vi "Check.vi"(7 "Address":string, 8 "Error In":errorcluster) -> (0 "Error Out":errorcluster)   [LabVIEW 2018, in "Tests.lvlib" / "Known Hosts.lvlib"]
uses:
  Known Hosts.lvlib
  src/Toolkit/Known Hosts/Type Definitions/Check Results.ctl
  <vilib>/Utility/error.llb/Clear Errors.vi
  src/Toolkit/Known Hosts/Support/Create from Session.vi
  <vilib>/Utility/sysdir.llb/Get System Directory.vi
  src/Toolkit/Known Hosts/Support/Destroy to Session.vi
  <vilib>/addons/_JKI Toolkits/Caraya/classes/Test/Test.lvclass
  <vilib>/addons/_JKI Toolkits/Caraya/classes/Assert/Assert.lvclass
  src/Toolkit/Known Hosts/Known Hosts.lvclass
  Tests.lvlib
  src/Toolkit/Session/Session.lvclass
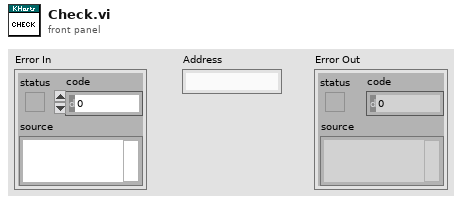
[diagram p1: front panel]
types:
  T1 = typedef "Toolkit.lvlib/Known Hosts.lvclass/Check Results.ctl" = i32
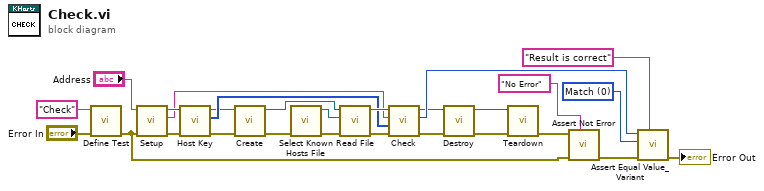
[diagram p0: block diagram]
diagram:
  w18 = T1 0 items=["Match", "Mismatch", "Not Found", "Failure"] ("Result")
  n1 = call <vilib>:"Define Test.vi"("error in (no error)"="Error In", "Label (VI Title)"="Check") -> ("error out"=w12:errorcluster)  [unwired: 9 in]
  n2 = call "Setup.vi"("Error In"=w12, "Address In"="Address") -> ("Error Out"=w13:errorcluster, "Address Out"=w10:string, "Sesssion"=w14:refnum<class "Session.lvclass">)  [unwired: 7 in]
  n3 = call "Host Key.vi"("Error In"=w13, "Session In"=w14) -> ("Error Out"=w1:errorcluster, "Host Key"=w15:u8[], "Sesssion Out"=w4:refnum<class "Session.lvclass">)  [unwired: 6 in, 1 out]
  n4 = call-poly "Create.vi"("Error In"=w1, "Session"=w4) -> ("Error Out"=w2:errorcluster, "Known Hosts"=w3:refnum<class "Known Hosts.lvclass">)  [unwired: 8 in]
  n5 = call "Select Known Hosts File.vi"("Error In"=w2) -> ("Error Out"=w24:errorcluster, "Known Hosts File"=w23:path)  [unwired: 9 in]
  n6 = call "Read File.vi"("Error In"=w24, "File"=w23, "Known Hosts In"=w3) -> ("Error Out"=w17:errorcluster, "Known Hosts Out"=w21:refnum<class "Known Hosts.lvclass">)  [unwired: 6 in, 1 out]
  n7 = call "Check.vi"("Error In"=w17, "Host Key"=w15, "Address"=w10, "Known Hosts In"=w21) -> ("Error Out"=w5:errorcluster, "Result"=w16:T1, "Known Hosts Out"=w8:refnum<class "Known Hosts.lvclass">)  [unwired: 5 in]
  n8 = call-poly "Destroy.vi"("Error In"=w5, "Known Hosts"=w8) -> ("Error Out"=w6:errorcluster, "Session"=w7:refnum<class "Session.lvclass">)  [unwired: 8 in]
  n9 = call "Teardown.vi"("Error In"=w6, "Session"=w7) -> ("Error Out"=w9:errorcluster)  [unwired: 9 in]
  n10 = call <vilib>:"Assert Not Error.vi"("Label"="No Error", "error in (no error)"=w12, "Not Error?"=w9) -> ("error out"=w22:errorcluster)  [unwired: 8 in]
  n11 = call <vilib>:"Assert Equal Value_Variant.vi"("Label"="Result is correct", "error in (no error)"=w22, "Y"=w18, "X"=w16) -> ("error out"=→"Error Out":errorcluster)  [unwired: 7 in]
